vi "Is an Actor-Interface.vi"(2 "Class in":refnum<vi>) -> (14 "Message Recipient Type":T1, 15 "Class out":refnum<vi>, 16 "Is Actor/Interface?":bool, 17 "AF Library FQN":string, 18 "Async AF Library FQN":string)   [LabVIEW 2023, in "Message Maker.lvclass"]
uses:
  Message Maker.lvclass
  Message Recipient Type.ctl
  Message Maker.lvclass/Message Maker.ctl
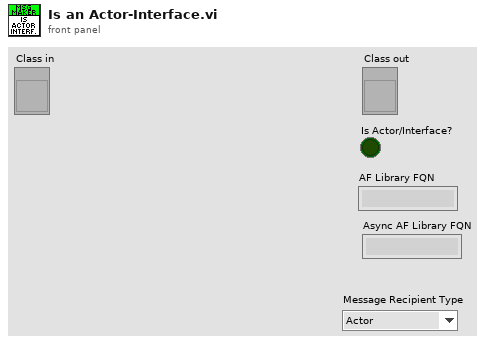
[diagram p1: front panel]
types:
  T1 = typedef "Message Maker.lvclass/Message Recipient Type.ctl" = enum16{"Actor", "Interface", "Async Actor"}
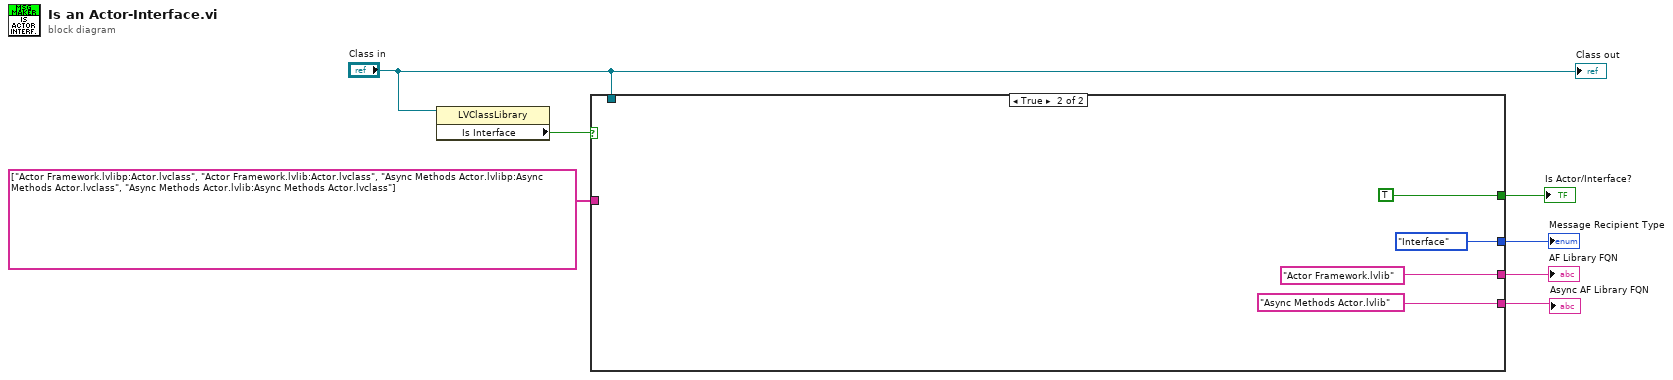
[diagram p0: block diagram]
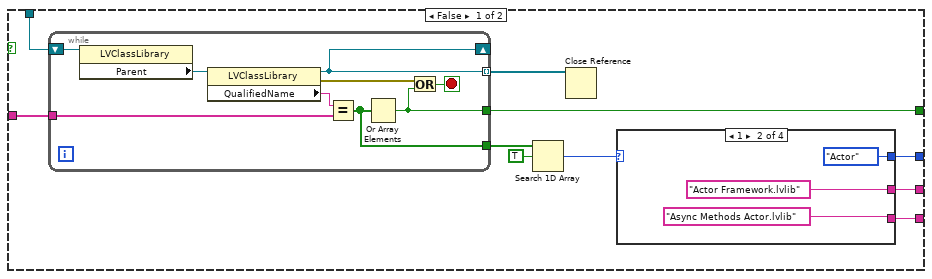
[diagram p2: hidden frame]
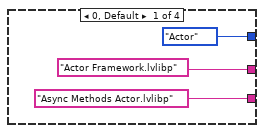
[diagram p3: hidden frame]
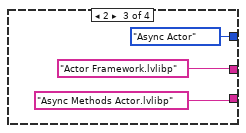
[diagram p4: hidden frame]
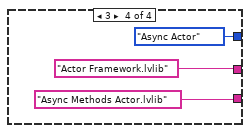
[diagram p5: hidden frame]
diagram:
  n1 = property class="LVClassLibrary"(reference="Class in") -> ("Is Interface"=w4:bool)  [unwired: 1 in, 2 out]
  n2 = case shown="True" w4 {
    tunnel: string[] ["Actor Framework.lvlibp:Actor.lvclass", "Actor Framework.lvlib:Actor.lvclass", "Async Methods Actor.lvlibp:Async Methods Actor.lvclass", "Async Methods Actor.lvlib:Async Methods Actor.lvclass"] -> [w17 _]
    tunnel: [w12 "Actor Framework.lvlib" ("Actor Class")] -> w6
    tunnel: "Class in" -> [w11 _]
    tunnel: [w10 TRUE] -> w3
    tunnel: [w9 Message_Recipient_Type."Interface" ("Message Recipient Type")] -> w2
    tunnel: [w8 "Async Methods Actor.lvlib" ("Actor Class")] -> w1
    frame False {
      n3 = while {
        shift-right: [w36] -> _
        shift-left: w11 -> [w38]
        tunnel: [w36] -> w16 mode=indexing
        tunnel: w17 -> [w34]
        tunnel: [w31] -> w10
        tunnel: [w30] -> w15
        stop <- w32 stop-if-true
        n4 = property class="LVClassLibrary"(reference=w38) -> ("Parent"=w37:refnum<vi>)  [unwired: 1 in, 2 out]
        n5 = property class="LVClassLibrary"(reference=w37) -> (reference out=w36:refnum<vi>, error out=w33:errorcluster, "QualifiedName"=w35:string)  [unwired: 1 in]
        n6 = Equal?(x=w35, y=w34) -> (x = y?=w30:bool[])
        n7 = Or Array Elements(Boolean array=w30) -> (logical OR=w31:bool)
        n8 = Or(x=w33, y=w31) -> (x .or. y?=w32:bool)
      }
      n9 = Search 1D Array(1D array=w15, element=TRUE) -> (index of element=w13:i32)  [unwired: 1 in]
      n10 = Close Reference(reference=w16) -> ()  [unwired: 1 in, 1 out]
      n11 = case shown="1" w13 {
        tunnel: ["Actor Framework.lvlibp" ("Actor Class") "Actor Framework.lvlib" ("Actor Class") "Actor Framework.lvlibp" ("Actor Class") "Actor Framework.lvlib" ("Actor Class")] -> w12
        tunnel: [Message_Recipient_Type."Actor" ("Message Recipient Type") Message_Recipient_Type."Actor" ("Message Recipient Type") Message_Recipient_Type."Async Actor" ("Message Recipient Type") Message_Recipient_Type."Async Actor" ("Message Recipient Type")] -> w9
        tunnel: ["Async Methods Actor.lvlibp" ("Actor Class") "Async Methods Actor.lvlib" ("Actor Class") "Async Methods Actor.lvlibp" ("Actor Class") "Async Methods Actor.lvlib" ("Actor Class")] -> w8
        frame 0, Default {
        }
        frame 1 {
        }
        frame 2 {
        }
        frame 3 {
        }
      }
    }
    frame True {
    }
  }
  "AF Library FQN" <- w6
  "Is Actor/Interface?" <- w3
  "Message Recipient Type" <- w2
  "Async AF Library FQN" <- w1
  "Class out" <- "Class in"
